vi "VM Spy - Dialog - History Info.vi"(8 "var name":string, 9 "vc handle":T3=-1) -> (2 "dup var name":string)   [LabVIEW 2021]
doc: "::: CalcExpress Toolkit :::\nCopyright (c) 2000-2026 Konstantin Shifershteyn. All rights reserved."
uses:
  vi.lib/addons/CalcExpress/cetypes.llb/VarMan Variable Context Handle.ctl
panel:
  out "save Eriter IDs":bool
  in  "enaWriterID":bool=TRUE caption="Save Writer IDs"
  out "has history":bool
  out "data type":u32(ring)=10 items=["String", "DBL Number", "identifier", "1D Array of DBL", "2D Array of DBL", "CDB Number", "1D Array of CDB", "2D Array of CDB", "1D Array of String", "2D Array of String", "Unknown data type"]
  out "oldest timestamp":dbl format="%<%H:%M:%S%2u  %d/%m/%Y>T"
  out "NewVals mode":T1 {"last read time" format="%<%H:%M:%S%2u  %d/%m/%Y>T"}
  out "update counter":u32
  out "newest timestamp":dbl format="%<%H:%M:%S%2u  %d/%m/%Y>T"
  out "stored values":u32
  in  "history length":u32 caption="history length (elements)"
  in  "value conditions":T2
  in  "time conditions":cluster{"Step, ms":u32, "Gate, ms":u32}
  in  "close":bool
  in  "config":bool
  in  "reset":bool
  in  "destroy":bool
  in  "create":bool
  out "Context":string
  out "Variable":string
  # "Configuration"
  # "Statistics"
  # "*) value conditions are only applicable if the Step parameter in the time conditions is greater than zero"
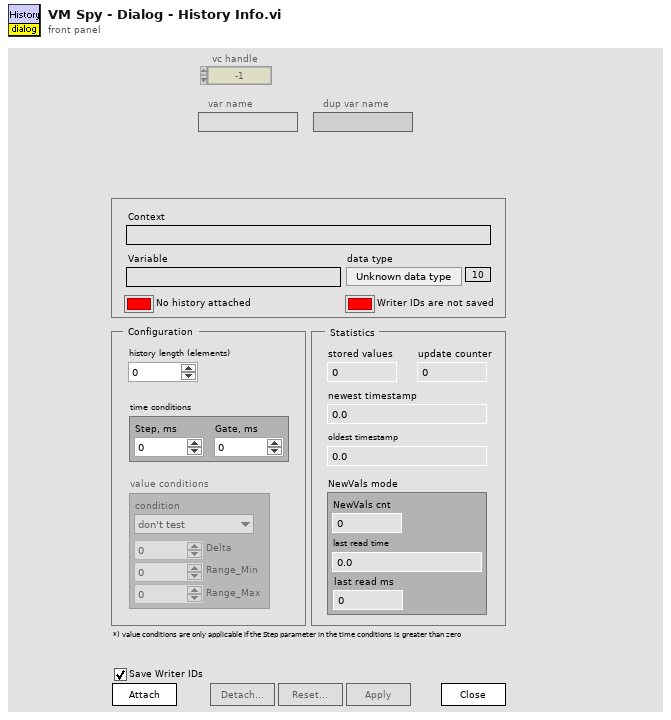
[diagram p1: front panel]
types:
  T1 = cluster{"NewVals cnt":u32, "last read time":dbl, "last read ms":u32}
  T2 = cluster{"condition":enum32{"don't test", "changed", "abs deviation", "rel deviation", "out of range", "within range"}, "Delta":dbl, "Range_Min":dbl, "Range_Max":dbl}
  T3 = typedef "VarMan Variable Context Handle.ctl" = i32
  T4 = typedef "VarMan History Info.ctl" = cluster{"var type":u32, "history length":u32, "stored values":u32, "update cnt":u32, "last update ms":u32, "newest timestamp":dbl, "oldest timestamp":dbl, "NewVals mode":cluster{"NewVals cnt":u32, "last read time":dbl, "last read ms":u32}, "time condition":cluster{"Step, ms":u32, "Gate, ms":u32}, "value condition":cluster{"condition":enum32{"don't test", "changed", "abs deviation", "rel deviation", "out of range", "within range"}, "Delta":dbl, "Range_Min":dbl, "Range_Max":dbl}}
  T5 = typedef "eventvkey.ctl" = enum16{"ASCII", "Enter", "Return", "Shift", "Ctrl", "Alt", "Cmd", "Opt", "Caps", "NumLock", "Clear", "Break", "Up", "Down", "Left", "Right", "Insert", "Delete", "Home", "End", "PageUp", "PageDown", "Escape", "Help", "Pause", "ScrollLock", "F1", "F2", "F3", "F4", "F5", "F6", "F7", "F8", "F9", "F10", "F11", "F12", "F13", "F14", "F15", "F16", "F17", "F18", "F19", "F20", "F21", "F22", "F23", "F24", "Play", "VolumeUp", "VolumeDown", "Mute", "Two Byte Char"}
  T6 = cluster{"Shift":bool, "Ctrl":bool, "Alt":bool, "Cmd":bool, "Opt":bool}
  T7 = enum32{"nop", "create", "destroy", "reset", "get info", "config", "create_wrid"}[]
  T8 = enum32{"nop", "create", "destroy", "reset", "get info", "config", "create_wrid"}
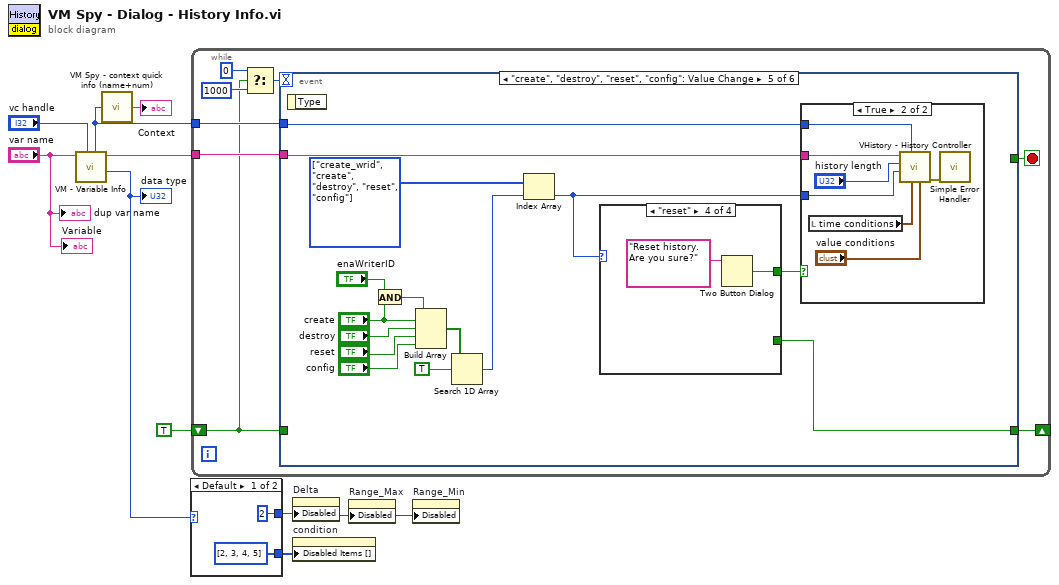
[diagram p0: block diagram]
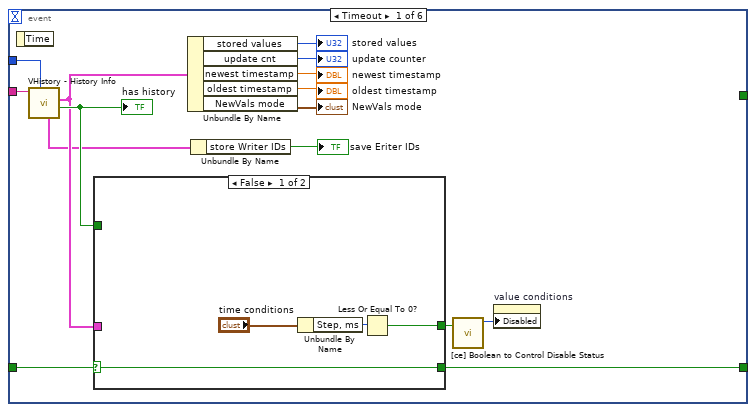
[diagram p2: hidden frame]
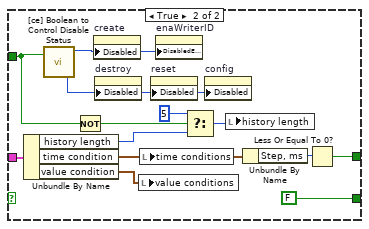
[diagram p3: hidden frame]
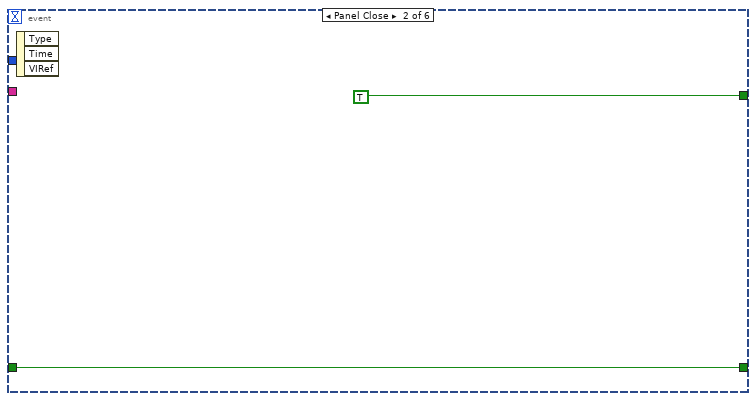
[diagram p4: hidden frame]
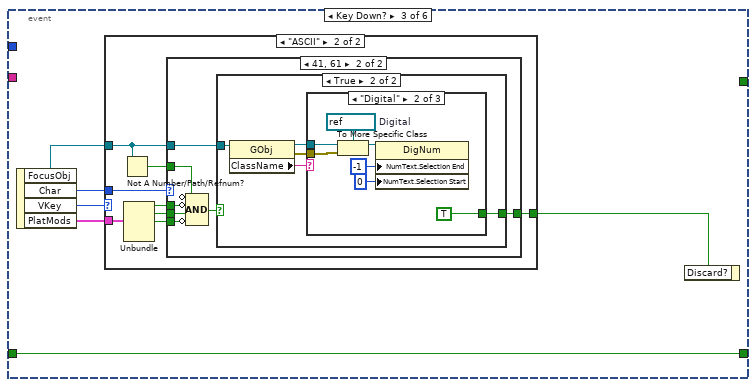
[diagram p5: hidden frame]
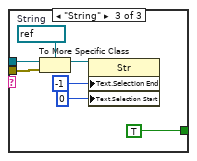
[diagram p10: hidden frame]
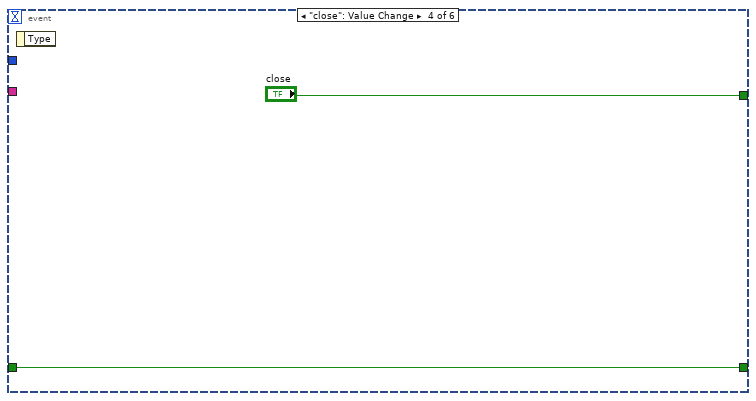
[diagram p11: hidden frame]
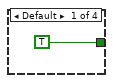
[diagram p12: hidden frame]
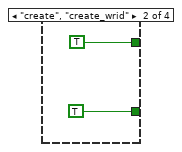
[diagram p13: hidden frame]
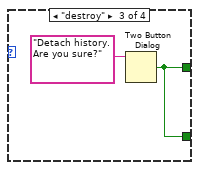
[diagram p14: hidden frame]
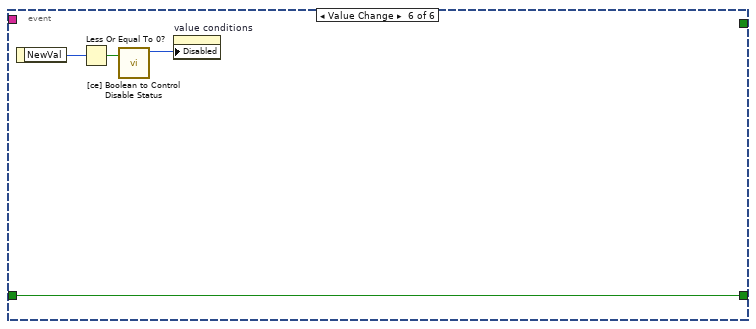
[diagram p16: hidden frame]
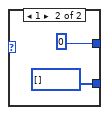
[diagram p17: hidden frame]
diagram:
  n1 = call "VM - Variable Info.vi"("VC Handle"="vc handle", "name_spec"="var name") -> ("var type"=w7:u32, "var name"=w3:string, "var VC Handle"=w2:T3)  [unwired: 4 in, 3 out]
  "data type" <- w7
  n2 = call "VM Spy - context quick info (name+num).vi"("handle"=w2) -> ("context info"=→"Context":string)  [unwired: 4 in]
  n3 = case shown="Default" w7 {
    tunnel: [u8 2 ("Disabled") u8 0 ("Disabled")] -> w6
    tunnel: [i32[] [2, 3, 4, 5] ("Disabled Items []") i32[] [] ("Disabled Items []")] -> w5
    frame Default {
    }
    frame 1 {
    }
  }
  n4 = while {
    tunnel: w3 -> [w21]
    tunnel: w2 -> [w20]
    shift-right: [w19] -> _
    shift-left: TRUE -> [w14]
    stop <- w18 stop-if-true
    n5 = Select(t=0, s=w14, f=1000) -> (s? t:f=w15:i32)
    n6 = event shown="[4] \"create\", \"destroy\", \"reset\", \"config\": Value Change" {
      selector: _ -> [_ _ _ _ _ _]
      dyn-events: _ -> [_ _ _ _ _ _]
      timeout: w15 -> [_ _ _ _ _ _]
      tunnel: w21 -> [w29 _ _ _ w106 _]
      tunnel: w20 -> [w28 _ _ _ w105 _]
      tunnel: w14 -> [w27 w54 w61 w96 _ w129]
      tunnel: [w26 w54 w61 w96 w98 w129] -> w19
      tunnel: [_ TRUE _ "close" _ _] -> w18
      event Timeout {
        n7 = event-data() -> ()  [unwired: 1 in, 1 out]
        n8 = call "VHistory - History Info.vi"("VC Handle"=w28, "name_spec"=w29) -> ("valid history"=w36:bool, "history info"=w35:T4, "more data"=w23:cluster{"store Writer IDs":bool})  [unwired: 5 in, 2 out]
        "has history" <- w36
        n9 = case shown="False" w27 {
          selector: w27 -> [w40 _]
          tunnel: w36 -> [_ w43]
          tunnel: w35 -> [_ w53]
          tunnel: [w40 FALSE] -> w26
          tunnel: [w37 w44] -> w25
          frame False {
            n10 = Unbundle By Name("time conditions") -> ("Step, ms"=w39:u32)
            n11 = Less Or Equal To 0?(x=w39) -> (x <= 0?=w37:bool)
          }
          frame True {
            n12 = Unbundle By Name(w53) -> ("history length"=w50:u32, "time condition"=w46:cluster{"Step, ms":u32, "Gate, ms":u32}, "value condition"=w52:T2)
            n13 = call "[ce] Boolean to Control Disable Status.vi"("Status in"=w43) -> ("Control Disable if True"=w42:u8, "Control Disable if False"=w41:u8)  [unwired: 3 in]
            n14 = Not(x=w43) -> (.not. x?=w49:bool)
            n15 = property on="create" class="Bool"("Disabled"=w42) -> ()  [unwired: 2 in, 2 out]
            n16 = property on="destroy" class="Bool"("Disabled"=w41) -> ()  [unwired: 2 in, 2 out]
            n17 = local write "value conditions"(w52) -> ()
            n18 = local write "time conditions"(w46) -> ()
            n19 = property on="reset" class="Bool"("Disabled"=w41) -> ()  [unwired: 2 in, 2 out]
            n20 = property on="enaWriterID" class="Bool (strict)"("DisabledEnum"=w42) -> ()  [unwired: 2 in, 2 out]
            n21 = Select(t=u32 5, s=w49, f=w50) -> (s? t:f=w47:u32)
            n22 = property on="config" class="Bool"("Disabled"=w41) -> ()  [unwired: 2 in, 2 out]
            n23 = local write "history length"(w47) -> ()
            n24 = Unbundle By Name(w46) -> ("Step, ms"=w45:u32)
            n25 = Less Or Equal To 0?(x=w45) -> (x <= 0?=w44:bool)
          }
        }
        n26 = Unbundle By Name(w35) -> ("stored values"=→"stored values":u32, "update cnt"=→"update counter":u32, "newest timestamp"=→"newest timestamp":dbl, "oldest timestamp"=→"oldest timestamp":dbl, "NewVals mode"=→"NewVals mode":T1)
        n27 = Unbundle By Name(w23) -> ("store Writer IDs"=→"save Eriter IDs":bool)
        n28 = call "[ce] Boolean to Control Disable Status.vi"("Status in"=w25) -> ("Control Disable if True"=w24:u8)  [unwired: 3 in, 1 out]
        n29 = property on="value conditions" class="Clust (strict)"("Disabled"=w24) -> ()  [unwired: 2 in, 2 out]
      }
      event Panel Close {
        n30 = event-data() -> ()  [unwired: 1 in, 3 out]
      }
      event Key Down? {
        n31 = event-data() -> ("FocusObj"=w56:refnum<vi>, "Char"=w57:i16, "VKey"=w58:T5, "PlatMods"=w59:T6)  [unwired: 1 in]
        n32 = case shown="\"ASCII\"" w58 {
          tunnel: w59 -> [_ w69]
          tunnel: [_ w63] -> w60
          tunnel: w57 -> [_ w65]
          tunnel: w56 -> [_ w64]
          frame Default {
          }
          frame "ASCII" {
            n33 = Not A Number/Path/Refnum?(number/path/refnum=w64) -> (NaN/Path/Refnum?=w62:bool)
            n34 = Unbundle(w69) -> ("Shift"=w68:bool, "Ctrl"=w67:bool, "Alt"=w66:bool)  [unwired: 2 out]
            n35 = case shown="41, 61" w65 {
              tunnel: w68 -> [_ w76]
              tunnel: w67 -> [_ w75]
              tunnel: w66 -> [_ w74]
              tunnel: w64 -> [_ w72]
              tunnel: [_ w71] -> w63
              tunnel: w62 -> [_ w70]
              frame Default {
              }
              frame 65, 97 {
                n36 = Compound Arithmetic op=AND(invert w70, invert w76, w75, invert w74) -> (w73:bool)
                n37 = case shown="True" w73 {
                  tunnel: w72 -> [_ w81]
                  tunnel: [_ w79] -> w71
                  frame False {
                  }
                  frame True {
                    n38 = property class="GObj"(reference=w81) -> (reference out=w78:refnum<vi>, error out=w77:errorcluster, "ClassName"=w80:string)  [unwired: 1 in]
                    n39 = case shown="\"Digital\"" w80 {
                      tunnel: [_ TRUE TRUE] -> w79
                      tunnel: w78 -> [_ w86 w93]
                      tunnel: w77 -> [_ w85 w92]
                      frame Default {
                      }
                      frame "Digital" {
                        w87 = refnum<vi> refnum  # Digital
                        n40 = To More Specific Class(target class=w87, reference=w86, error in=w85) -> (specific class reference=w84:refnum<vi>)  [unwired: 1 out]
                        n41 = property class="DigNum"(reference=w84, "NumText.Selection End"=-1 ("Numeric Text.Selection:End"), "NumText.Selection Start"=u32 0 ("Numeric Text.Selection:Start")) -> ()  [unwired: 1 in, 2 out]
                      }
                      frame "String" {
                        w94 = refnum<vi> refnum  # String
                        n42 = To More Specific Class(target class=w94, reference=w93, error in=w92) -> (specific class reference=w91:refnum<vi>)  [unwired: 1 out]
                        n43 = property class="Str"(reference=w91, "Text.Selection End"=-1 ("Numeric Text.Selection:End"), "Text.Selection Start"=u32 0 ("Numeric Text.Selection:Start")) -> ()  [unwired: 1 in, 2 out]
                      }
                    }
                  }
                }
              }
            }
          }
        }
        n44 = event-data("Discard?"=w60) -> ()  [unwired: 1 in, 1 out]
      }
      event "close": Value Change {
        n45 = event-data() -> ()  [unwired: 1 in, 1 out]
      }
      event "create", "destroy", "reset", "config": Value Change {
        w112 = T7 [enum."create_wrid", enum."create", enum."destroy", enum."reset", enum."config"] items=["nop", "create", "destroy", "reset", "get info", "config", "create_wrid"]
        n46 = event-data() -> ()  [unwired: 1 in, 1 out]
        n47 = And(x="enaWriterID", y="create") -> (x .and. y?=w100:bool)
        n48 = Build Array(w100, "create", "destroy", "reset", "config") -> (w110:bool[])
        n49 = Search 1D Array(1D array=w110, element=TRUE) -> (index of element=w104:i32)  [unwired: 1 in]
        n50 = Index Array(array=w112, index=w104) -> (element=w99:T8)
        n51 = case shown="\"reset\"" w99 {
          tunnel: [TRUE TRUE w116 w119] -> w103
          tunnel: [_ TRUE w116 _] -> w98
          frame Default {
          }
          frame "create", "create_wrid" {
          }
          frame "destroy" {
            n52 = Two Button Dialog(message="Detach history. Are you sure?") -> (T button?=w116:bool)  [unwired: 2 in]
          }
          frame "reset" {
            n53 = Two Button Dialog(message="Reset history. Are you sure?") -> (T button?=w119:bool)  [unwired: 2 in]
          }
        }
        n54 = case shown="True" w103 {
          tunnel: w106 -> [_ w126]
          tunnel: w105 -> [_ w125]
          tunnel: w99 -> [_ w120]
          frame False {
          }
          frame True {
            n55 = local read "time conditions"() -> (w121:cluster{"Step, ms":u32, "Gate, ms":u32})
            n56 = call "VHistory - History Controller.vi"("value condition"="value conditions", "time conditions"=w121, "VC Handle"=w125, "cmd (nop:default)"=w120, "history length"="history length", "name_spec"=w126) -> ("error out"=w124:errorcluster)  [unwired: 2 in, 3 out]
            n57 = call <vilib>:"Simple Error Handler.vi"("error in (no error)"=w124) -> ()  [unwired: 4 in, 5 out]
          }
        }
      }
      event "time conditions.Step, ms": Value Change {
        n58 = event-data() -> ("NewVal"=w130:u32)  [unwired: 1 in]
        n59 = Less Or Equal To 0?(x=w130) -> (x <= 0?=w128:bool)
        n60 = call "[ce] Boolean to Control Disable Status.vi"("Status in"=w128) -> ("Control Disable if True"=w127:u8)  [unwired: 3 in, 1 out]
        n61 = property on="value conditions" class="Clust (strict)"("Disabled"=w127) -> ()  [unwired: 2 in, 2 out]
      }
    }
  }
  n62 = property on="Delta" class="DigNum (strict)"("Disabled"=w6) -> ()  [unwired: 2 in, 2 out]
  n63 = property on="condition" class="Enum (strict)"("Disabled Items []"=w5) -> ()  [unwired: 2 in, 2 out]
  n64 = property on="Range_Max" class="DigNum (strict)"("Disabled"=w6) -> ()  [unwired: 2 in, 2 out]
  n65 = property on="Range_Min" class="DigNum (strict)"("Disabled"=w6) -> ()  [unwired: 2 in, 2 out]
  "dup var name" <- "var name"
  "Variable" <- "var name"
